vi "InsertMoney.vi"(8 "error in (no error)":errorcluster, 11 "object in":refnum<class "NoMoneyState.lvclass">) -> (0 "error out":errorcluster, 3 "object out":refnum<class "State.lvclass">)   [LabVIEW 2020, in "NoMoneyState.lvclass"]
uses:
  NoMoneyState.lvclass
  State_class/State.lvclass
  HasMoneyState_class/HasMoneyState.lvclass
  C:/Projects/OpenGDS_DesignPatterns/State1/State_class/State.lvclass
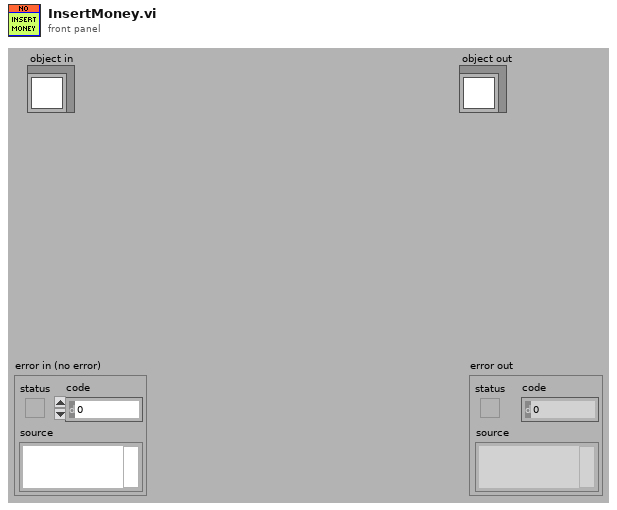
[diagram p1: front panel]
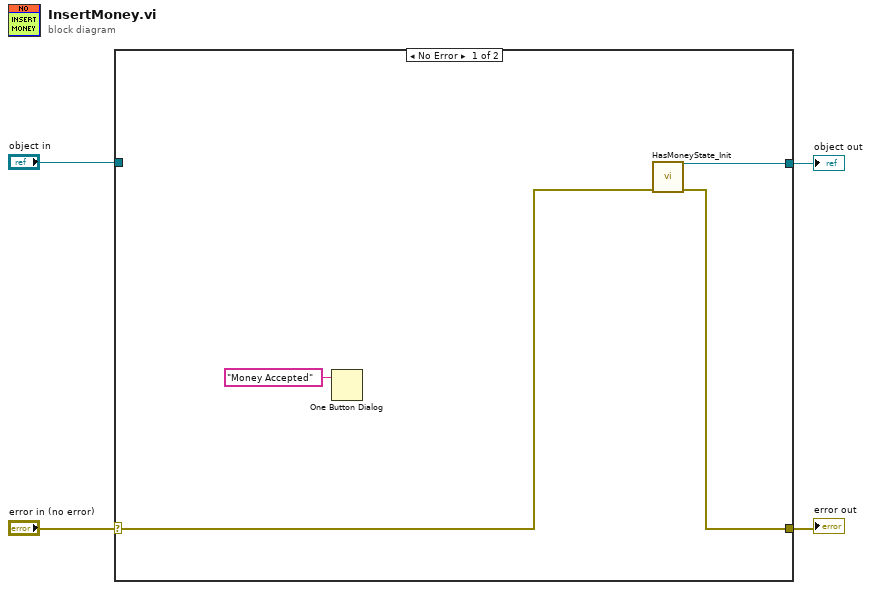
[diagram p0: block diagram]
diagram:
  n1 = case shown="No Error" "error in (no error)" {
    selector: "error in (no error)" -> [w6 w9]
    tunnel: [w5 w9] -> w3
    tunnel: [w7 _] -> w1
    tunnel: "object in" -> [_ _]
    frame No Error {
      n2 = One Button Dialog(message="Money Accepted" ("TextIn")) -> ()  [unwired: 1 in, 1 out]
      n3 = call "HasMoneyState_Init.vi"("error in (no error)"=w6) -> ("error out"=w5:errorcluster, "object out"=w7:refnum<class "HasMoneyState.lvclass">)  [unwired: 9 in]
    }
    frame Error {
    }
  }
  "error out" <- w3
  "object out" <- w1
